vi "Callee2.vi"(0 "x":dbl) -> (1 "y":dbl)   [LabVIEW 2026]
doc: "Probe fixture: y is x plus 2."
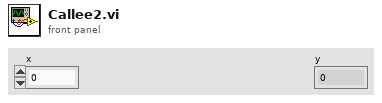
[diagram p1: front panel]
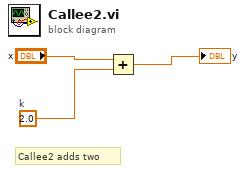
[diagram p0: block diagram]
diagram:
  w2 = 2.0  # k
  # "Callee2 adds two"
  n1 = Add(x="x", y=w2) -> (x+y=→"y":dbl)
